vi "StateUpdate.vi"(8 "error in (no error)":errorcluster, 11 "View in":refnum<class "View.lvclass">) -> (0 "error out":errorcluster, 3 "View out":refnum<class "View.lvclass">)   [LabVIEW 2024, in "View.lvclass"]
uses:
  View.lvclass
  View.lvclass/View.ctl
  Viewmodel/Viewmodel.lvclass
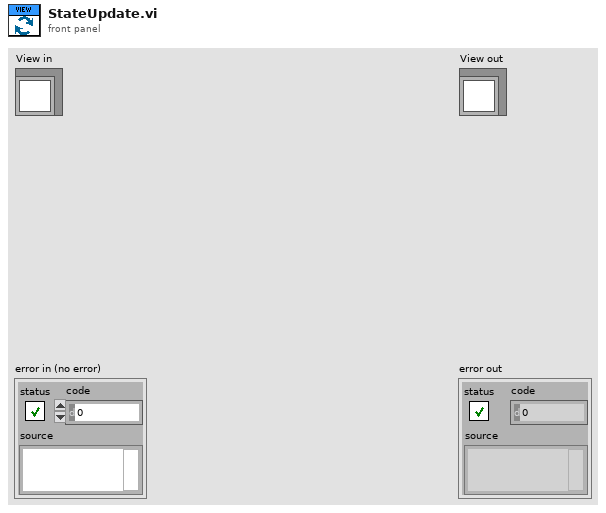
[diagram p1: front panel]
types:
  T1 = typedef "View.lvclass/UIRefs.ctl" = cluster{"Counter":refnum<vi>, "Increment":refnum<vi>, "Decrement":refnum<vi>}
  T2 = typedef "Viewmodel.lvclass/State.ctl" = cluster{"Counter":i32}
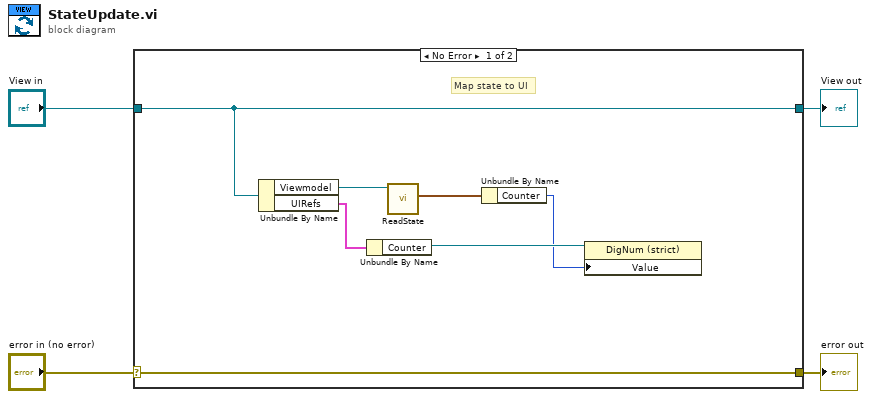
[diagram p0: block diagram]
diagram:
  n1 = case shown="No Error" "error in (no error)" {
    selector: "error in (no error)" -> [w11 w13]
    tunnel: [w11 w13] -> w3
    tunnel: [w10 w12] -> w1
    tunnel: "View in" -> [w10 w12]
    frame No Error {
      # "Map state to UI"
      n2 = Unbundle By Name(w10) -> ("Viewmodel"=w7:refnum<class "Viewmodel.lvclass">, "UIRefs"=w9:T1)
      n3 = Unbundle By Name(w9) -> ("Counter"=w8:refnum<vi>)
      n4 = call "ReadState.vi"("Viewmodel in"=w7) -> ("State"=w6:T2)  [unwired: 8 in, 2 out]
      n5 = Unbundle By Name(w6) -> ("Counter"=w5:i32)
      n6 = property class="DigNum (strict)"(reference=w8, "Value"=w5) -> ()  [unwired: 1 in, 2 out]
    }
    frame Error {
    }
  }
  "error out" <- w3
  "View out" <- w1
